vi "ActiveObjects_DynamicEvents_ProcessRepository_Native.vi"(0 "reference in":refnum<class>, 1 "Action(ReadRepository)":T1(ring), 5 "Error In":errorcluster) -> (7 "QueueFromProcess":refnum<queue>, 9 "ProcessViRef":refnum<vi>, 11 "ProcessSyncQueue":refnum<queue>, 13 "EventFromProcess":refnum<user-event>, 14 "reference out":refnum<class>, 15 "EventsToProcess":refnum<user-event>, 17 "ProcessAlreadyStarted":bool, 19 "Error Out":errorcluster)   [LabVIEW 2020]
uses:
  ActiveObjects_DynamicEvents_Process.ctl
panel:
  # "Use this indicator for sending messages to the Process VI"
  # "These indicators are used by the process VIs"
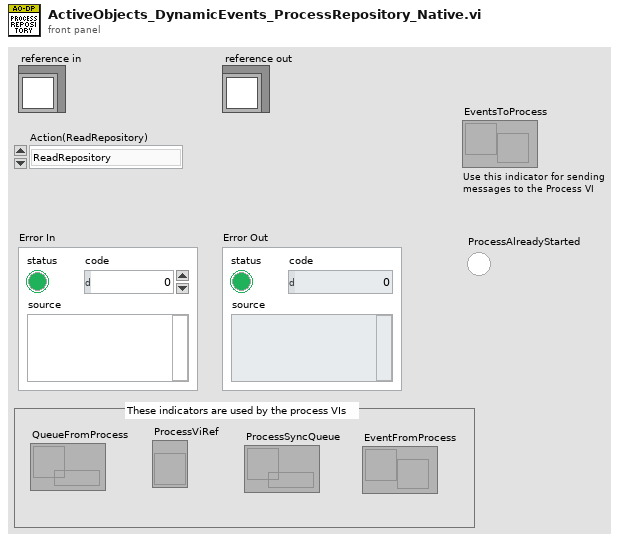
[diagram p1: front panel]
types:
  T1 = enum16{"ReadRepository", "CreateNew", "CreateOrLookUpExisting", "ReadRepositoryAndDestroy"}
  T2 = typedef "ActiveObjects_DynamicEvents_Process.ctl" = cluster{"EventsToProcess":refnum<user-event>, "EventFromProcess":refnum<user-event>, "ProcessSyncQueue":refnum<queue>, "ProcessViRef":refnum<vi>, "QueueFromProcess":refnum<queue>}
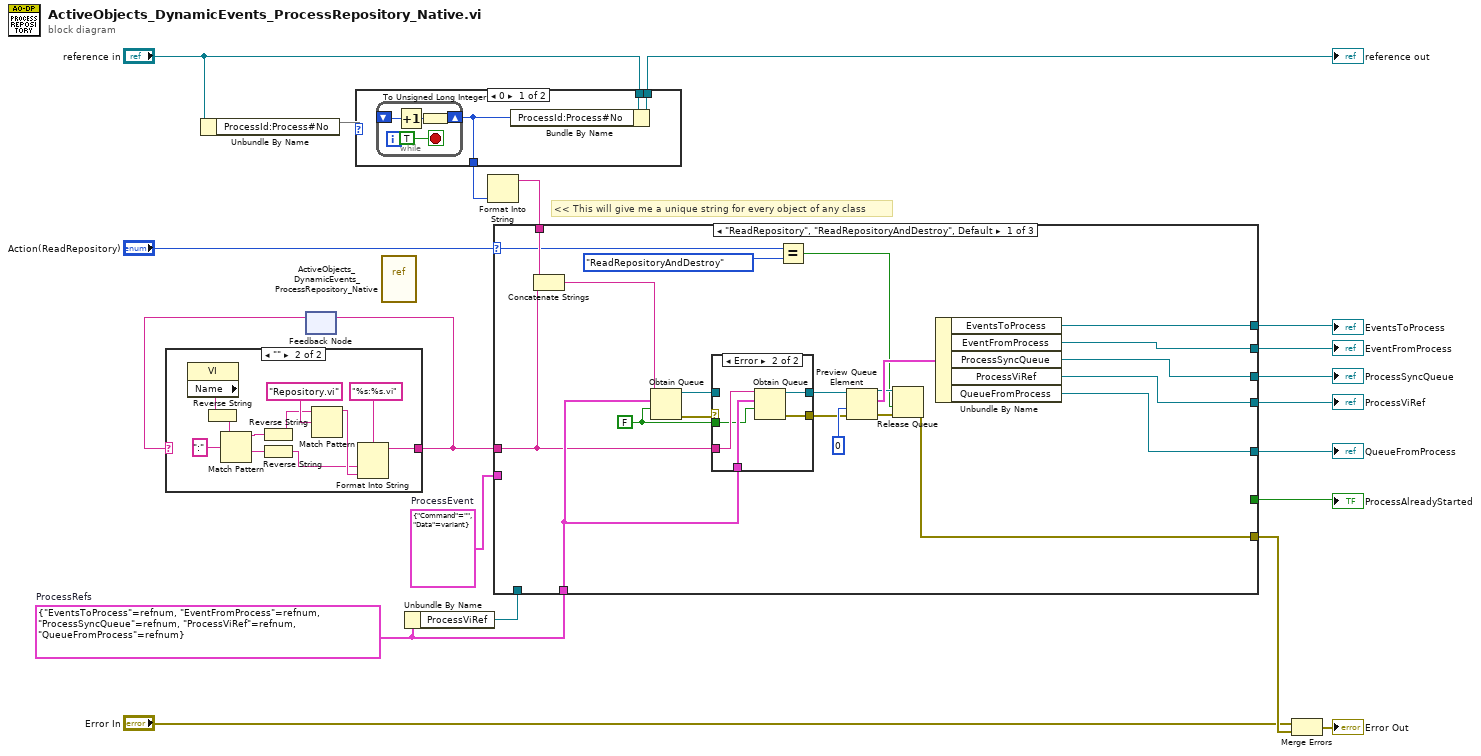
[diagram p0: block diagram]
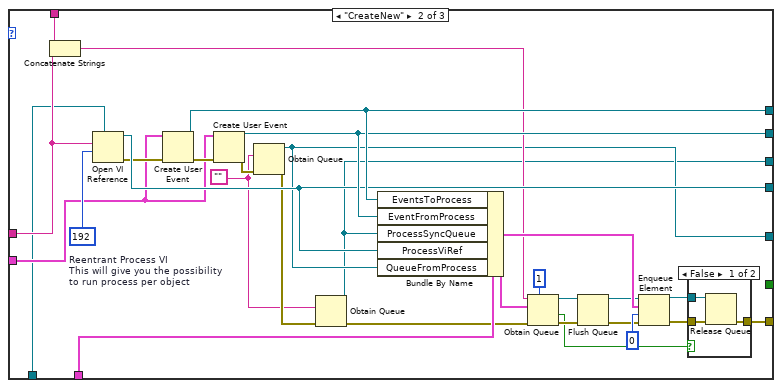
[diagram p5: hidden frame]
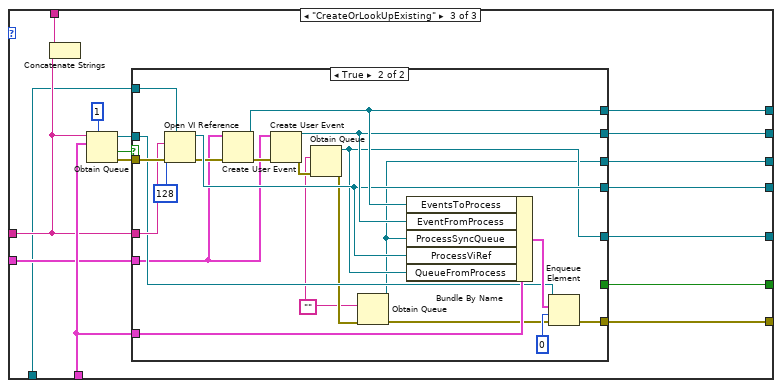
[diagram p7: hidden frame]
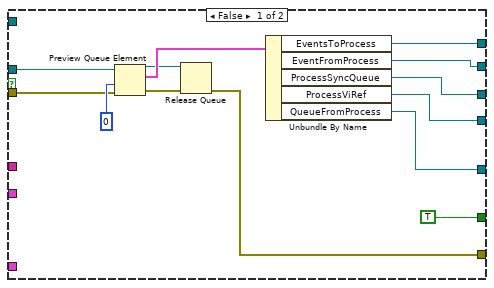
[diagram p8: hidden frame]
diagram:
  w1 = T2 {"EventsToProcess"=refnum, "EventFromProcess"=refnum, "ProcessSyncQueue"=refnum, "ProcessViRef"=refnum, "QueueFromProcess"=refnum}  # ProcessRefs
  w7 = cluster{"Command":string, "Data":variant} {"Command"="", "Data"=variant}  # ProcessEvent
  # "<< This will give me a unique string for every object of any class"
  n1 = Unbundle By Name("reference in") -> ("ProcessId:Process#No"=w11)
  n2 = feedback #1() -> (w4:string)  [unwired: 1 in]
  n3 = case shown="\"\"" w4 {
    selector: w4 -> [w21 _]
    tunnel: [w21 w22] -> w5
    frame Default {
    }
    frame "" {
      n4 = property class="VI"() -> ("Name"=w24:string)  [unwired: 2 in, 2 out]
      n5 = Reverse String(1:w24) -> (0:w25:string)
      n6 = Match Pattern(string=w25, regular expression=":") -> (before substring=w29:string, after substring=w26:string)  [unwired: 1 in, 2 out]
      n7 = Reverse String(1:w29) -> (0:w30:string)
      n8 = Reverse String(1:w26) -> (0:w28:string)
      n9 = Match Pattern(string=w30, regular expression="Repository.vi") -> (before substring=w32:string)  [unwired: 1 in, 3 out]
      n10 = Format Into String(format string="%s:%s.vi", w28, w32) -> (resulting string=w22:string)  [unwired: 2 in, 1 out]
    }
  }
  n11 = feedback-in #1(w5) -> ()
  n12 = case shown="0" w11 {
    selector: w11 -> [_ w41]
    tunnel: [w33 w41] -> w12
    tunnel: "reference in" -> [w35 w40]
    tunnel: [w34 w40] -> w9
    frame 0 {
      n13 = while {
        shift-right: [w36] -> w33
        shift-left: _ -> [w38]
        stop <- TRUE stop-if-true
        n14 = Increment(x=w38) -> (x+1=w37:u32)
        n15 = To Unsigned Long Integer(number=w37) -> (unsigned 32bit integer=w36:u32)
      }
      n16 = Bundle By Name(cluster=w35, "ProcessId:Process#No"=w33) -> (w34:refnum<class>)
    }
    frame Default {
    }
  }
  "reference out" <- w9
  n17 = vi-ref "ActiveObjects_DynamicEvents_ProcessRepository_Native.vi"() -> ()  [unwired: 1 out]
  n18 = Unbundle By Name(w1) -> ("ProcessViRef"=w3:refnum<vi>)
  n19 = Format Into String(w12) -> (resulting string=w8:string)  [unwired: 3 in, 1 out]
  n20 = case shown="\"ReadRepository\", \"ReadRepositoryAndDestroy\", Default" "Action(ReadRepository)" {
    selector: "Action(ReadRepository)" -> [w43 _ _]
    tunnel: [w59 w79 w117] -> w19
    tunnel: [w61 w99 w119] -> w17
    tunnel: [w60 w98 w118] -> w18
    tunnel: [w62 w97 w116] -> w16
    tunnel: w1 -> [w54 w89 w112]
    tunnel: w8 -> [w52 w88 w108]
    tunnel: [w45 w72 w115] -> w15
    tunnel: w5 -> [w51 w86 w105]
    tunnel: [_ _ w110] -> w14
    tunnel: w7 -> [_ w85 w107]
    tunnel: [w49 w83 w106] -> w6
    tunnel: w3 -> [_ w71 w104]
    frame "ReadRepository", "ReadRepositoryAndDestroy", Default {
      w53 = FALSE ("create if not found? (T)")
      n21 = Concatenate Strings(w52, w51) -> (w50:string)
      n22 = Obtain Queue(name (unnamed)=w50, element data type=w54, create if not found? (T)=w53) -> (queue out=w56:refnum<queue>, error out=w58:errorcluster)  [unwired: 2 in, 1 out]
      n23 = case shown="Error" w58 {
        selector: w58 -> [w65 _]
        tunnel: [w65 w67] -> w57
        tunnel: w56 -> [w64 _]
        tunnel: [w64 w68] -> w55
        tunnel: w54 -> [_ w70]
        tunnel: w51 -> [_ w69]
        tunnel: w53 -> [_ w66]
        frame No Error {
        }
        frame Error {
          n24 = Obtain Queue(name (unnamed)=w69, element data type=w70, create if not found? (T)=w66) -> (queue out=w68:refnum<queue>, error out=w67:errorcluster)  [unwired: 2 in, 1 out]
        }
      }
      n25 = Equal?(x=w43, y=T1."ReadRepositoryAndDestroy") -> (x = y?=w42:bool)
      n26 = Preview Queue Element(queue=w55, timeout in ms (-1)=0, error in (no error)=w57) -> (queue out=w47:refnum<queue>, element=w48:T2, error out=w46:errorcluster)  [unwired: 1 out]
      n27 = Release Queue(queue=w47, force destroy? (F)=w42, error in (no error)=w46) -> (error out=w45:errorcluster)  [unwired: 2 out]
      n28 = Unbundle By Name(w48) -> ("EventsToProcess"=w61:refnum<user-event>, "EventFromProcess"=w60:refnum<user-event>, "ProcessSyncQueue"=w59:refnum<queue>, "ProcessViRef"=w62:refnum<vi>, "QueueFromProcess"=w49:refnum<queue>)
    }
    frame "CreateNew" {
      w80 = ""
      w94 = 192  # Reentrant Process VI This will give you the possibility to run process per object
      n29 = Concatenate Strings(w88, w86) -> (w87:string)
      n30 = Open VI Reference(type specifier VI Refnum (for type only)=w71, vi path=w86, options=w94) -> (vi reference=w97:refnum<vi>, error out=w95:errorcluster)  [unwired: 3 in]
      n31 = Create User Event(user event datatype=w85, error in=w95) -> (user event=w99:refnum<user-event>, error out=w96:errorcluster)
      n32 = Create User Event(user event datatype=w85, error in=w96) -> (user event=w98:refnum<user-event>, error out=w84:errorcluster)
      n33 = Obtain Queue(element data type=w80, error in (no error)=w84) -> (queue out=w83:refnum<queue>, error out=w82:errorcluster)  [unwired: 3 in, 1 out]
      n34 = Obtain Queue(element data type=w80, error in (no error)=w82) -> (queue out=w79:refnum<queue>, error out=w81:errorcluster)  [unwired: 3 in, 1 out]
      n35 = Bundle By Name(cluster=w89, "EventsToProcess"=w99, "EventFromProcess"=w98, "ProcessSyncQueue"=w79, "ProcessViRef"=w97, "QueueFromProcess"=w83) -> (w92:T2)
      n36 = Obtain Queue(max queue size (-1, unlimited)=1, name (unnamed)=w87, element data type=w92, error in (no error)=w81) -> (queue out=w93:refnum<queue>, created new?=w75:bool, error out=w77:errorcluster)  [unwired: 1 in]
      n37 = Flush Queue(queue=w93, error in (no error)=w77) -> (queue out=w78:refnum<queue>, error out=w76:errorcluster)  [unwired: 1 out]
      n38 = Enqueue Element(queue=w78, element=w92, timeout in ms (-1)=0, error in (no error)=w76) -> (queue out=w73:refnum<queue>, error out=w74:errorcluster)  [unwired: 1 out]
      n39 = case shown="False" w75 {
        tunnel: w74 -> [w102 w103]
        tunnel: w73 -> [w101 _]
        tunnel: [w100 w103] -> w72
        frame False {
          n40 = Release Queue(queue=w101, error in (no error)=w102) -> (error out=w100:errorcluster)  [unwired: 1 in, 2 out]
        }
        frame True {
        }
      }
    }
    frame "CreateOrLookUpExisting" {
      n41 = Concatenate Strings(w108, w105) -> ()  [unwired: 1 out]
      n42 = Obtain Queue(max queue size (-1, unlimited)=1, name (unnamed)=w105, element data type=w112) -> (queue out=w113:refnum<queue>, created new?=w114:bool, error out=w111:errorcluster)  [unwired: 2 in]
      n43 = case shown="True" w114 {
        tunnel: [w132 w153] -> w119
        tunnel: [w131 w152] -> w118
        tunnel: [w130 w136] -> w117
        tunnel: [w129 w151] -> w116
        tunnel: [w120 w150] -> w115
        tunnel: w112 -> [_ w149]
        tunnel: w111 -> [w126 w144]
        tunnel: w105 -> [_ w143]
        tunnel: w113 -> [w127 w142]
        tunnel: [TRUE _] -> w110
        tunnel: w107 -> [_ w141]
        tunnel: [w123 w139] -> w106
        tunnel: w104 -> [_ w134]
        frame False {
          n44 = Preview Queue Element(queue=w127, timeout in ms (-1)=0, error in (no error)=w126) -> (queue out=w122:refnum<queue>, element=w125:T2, error out=w121:errorcluster)  [unwired: 1 out]
          n45 = Release Queue(queue=w122, error in (no error)=w121) -> (error out=w120:errorcluster)  [unwired: 1 in, 2 out]
          n46 = Unbundle By Name(w125) -> ("EventsToProcess"=w132:refnum<user-event>, "EventFromProcess"=w131:refnum<user-event>, "ProcessSyncQueue"=w130:refnum<queue>, "ProcessViRef"=w129:refnum<vi>, "QueueFromProcess"=w123:refnum<queue>)
        }
        frame True {
          w137 = ""
          n47 = Open VI Reference(type specifier VI Refnum (for type only)=w134, vi path=w143, options=128, error in (no error)=w144) -> (vi reference=w151:refnum<vi>, error out=w147:errorcluster)  [unwired: 2 in]
          n48 = Create User Event(user event datatype=w141, error in=w147) -> (user event=w153:refnum<user-event>, error out=w148:errorcluster)
          n49 = Create User Event(user event datatype=w141, error in=w148) -> (user event=w152:refnum<user-event>, error out=w140:errorcluster)
          n50 = Obtain Queue(element data type=w137, error in (no error)=w140) -> (queue out=w139:refnum<queue>, error out=w138:errorcluster)  [unwired: 3 in, 1 out]
          n51 = Obtain Queue(element data type=w137, error in (no error)=w138) -> (queue out=w136:refnum<queue>, error out=w135:errorcluster)  [unwired: 3 in, 1 out]
          n52 = Bundle By Name(cluster=w149, "EventsToProcess"=w153, "EventFromProcess"=w152, "ProcessSyncQueue"=w136, "ProcessViRef"=w151, "QueueFromProcess"=w139) -> (w146:T2)
          n53 = Enqueue Element(queue=w142, element=w146, timeout in ms (-1)=0, error in (no error)=w135) -> (error out=w150:errorcluster)  [unwired: 2 out]
        }
      }
    }
  }
  "ProcessSyncQueue" <- w19
  "EventsToProcess" <- w17
  "EventFromProcess" <- w18
  "ProcessViRef" <- w16
  "ProcessAlreadyStarted" <- w14
  "QueueFromProcess" <- w6
  n54 = Merge Errors("Error In", w15) -> (→"Error Out":errorcluster)
